vi "OPC Show.vi"(7 "queue array in":refnum<queue>[](array[refnum]), 8 "Value":variant[](array[variant]), 9 "Read":u8[](array[numeric]), 11 "Ctl In":refnum<vi>[](array[refnum])) -> ()   [LabVIEW 2012]
uses:
  <vilib>/Utility/miscctls.llb/LVRowAndColumnTypeDef.ctl
  Queue VIs/Type define/element data type.ctl
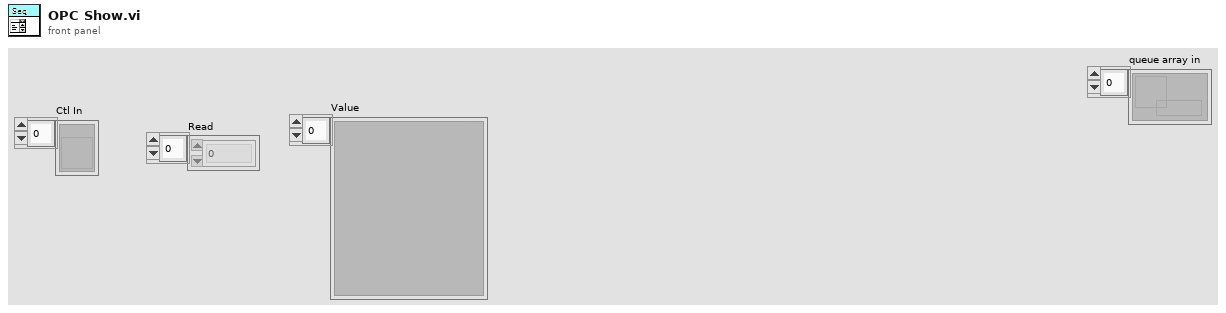
[diagram p1: front panel]
types:
  T1 = typedef "LVRowAndColumnTypeDef.ctl" = cluster{"Row":i32, "Column":i32}
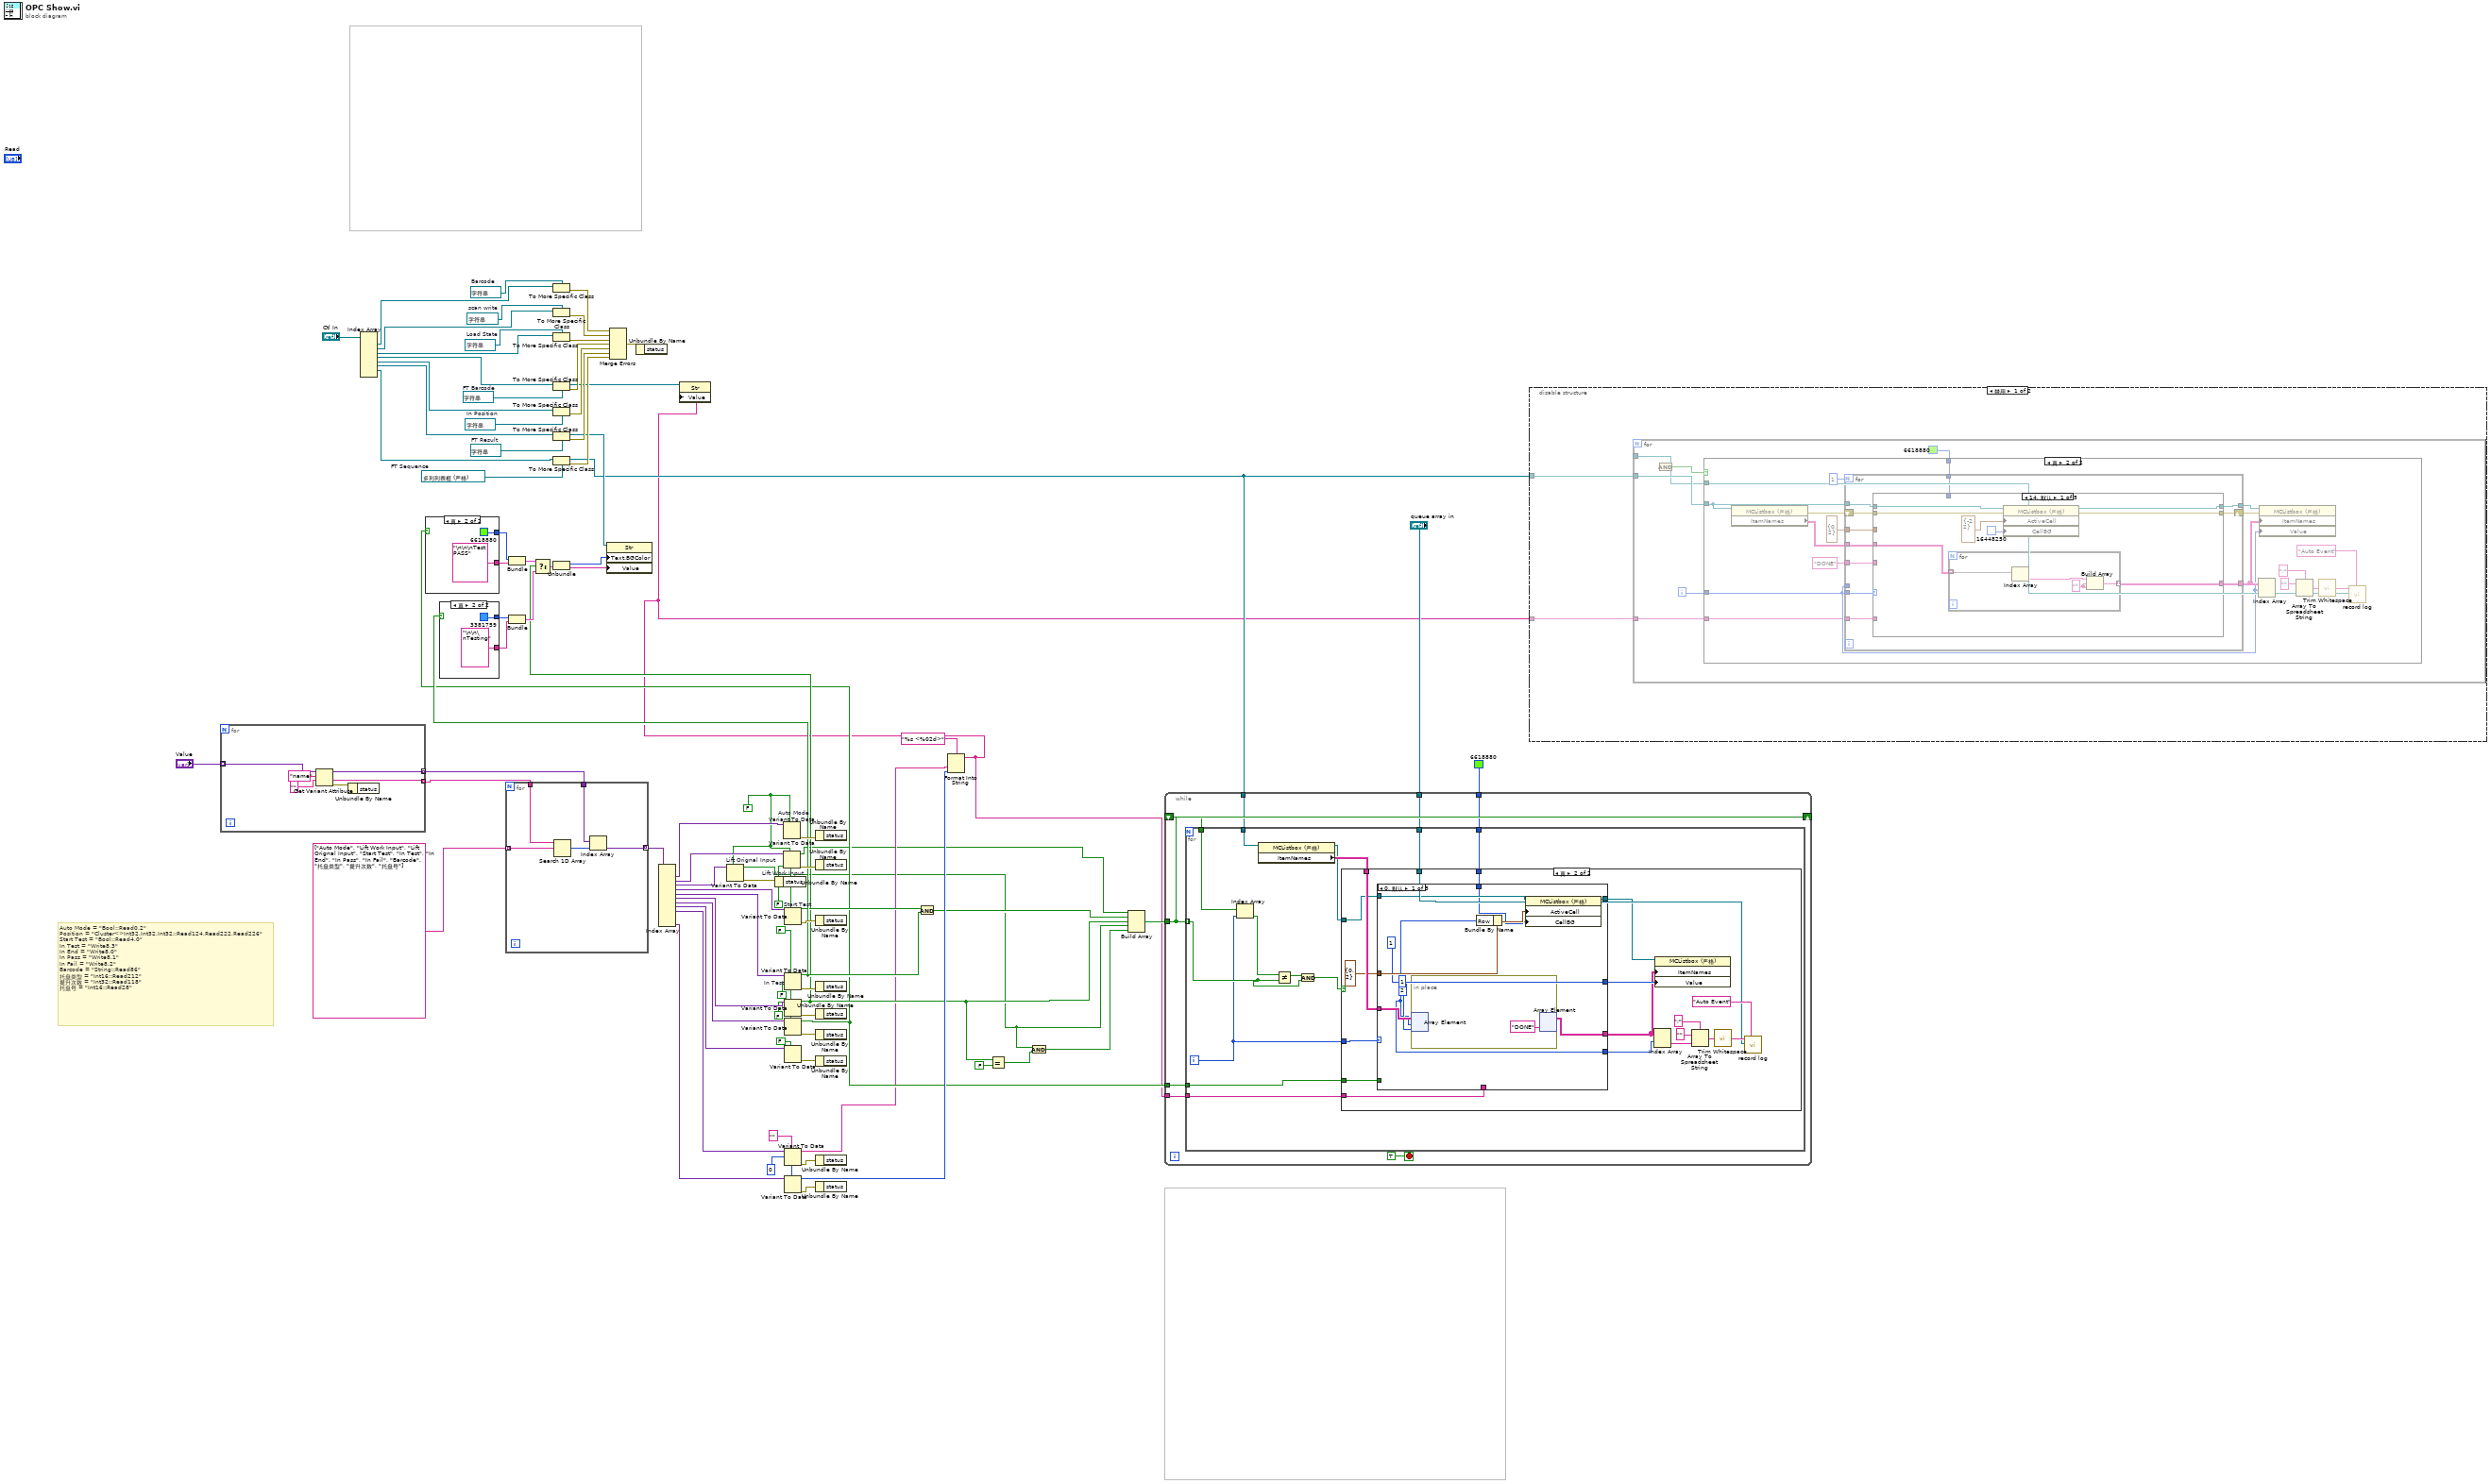
[diagram p0: block diagram]
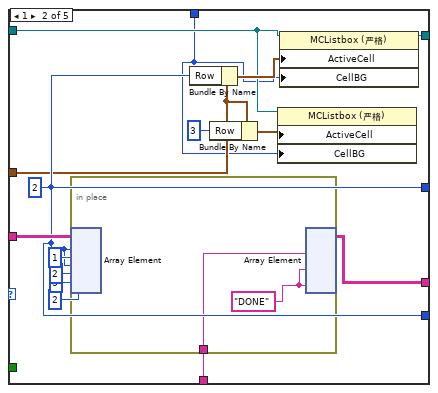
[diagram p3: hidden frame]
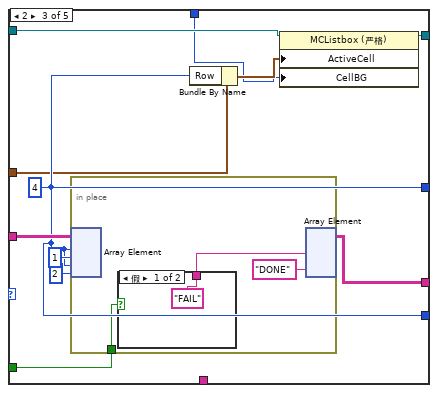
[diagram p4: hidden frame]
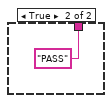
[diagram p5: hidden frame]
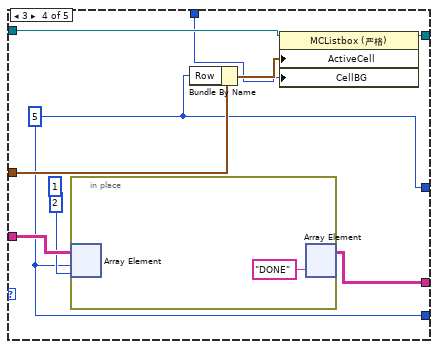
[diagram p6: hidden frame]
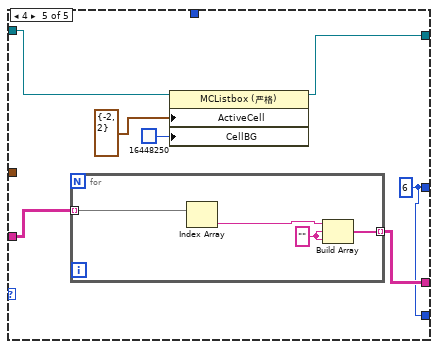
[diagram p7: hidden frame]
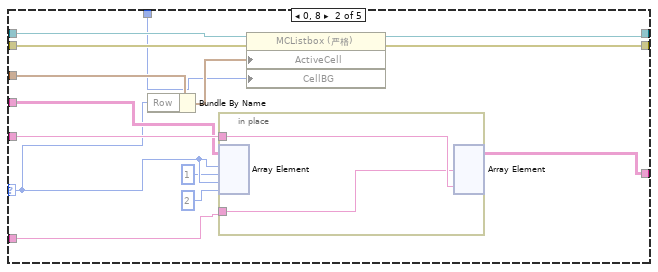
[diagram p9: hidden frame]
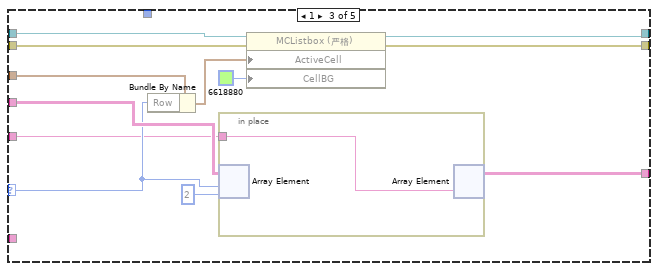
[diagram p10: hidden frame]
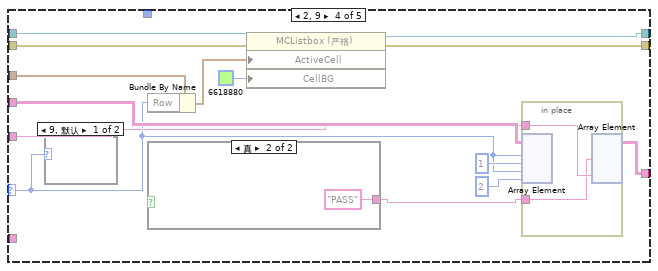
[diagram p11: hidden frame]
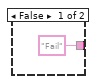
[diagram p13: hidden frame]
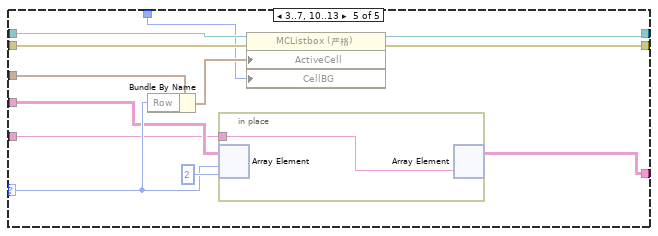
[diagram p14: hidden frame]
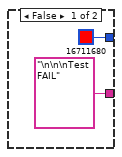
[diagram p16: hidden frame]
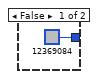
[diagram p17: hidden frame]
diagram:
  w4 = FALSE
  w77 = refnum<vi> refnum  # FT Sequence
  w78 = refnum<vi> refnum  # FT Result
  w79 = refnum<vi> refnum  # In Position
  w80 = refnum<vi> refnum  # FT Barcode
  w81 = refnum<vi> refnum  # Load State
  w82 = refnum<vi> refnum  # scan write
  w83 = refnum<vi> refnum  # Barcode
  # "Auto Mode = \"Bool::Read0.2\"\nPosition = \"Cluster<>Int32,Int32,Int32::Read124,Read222,Read226\"\nStart Test = \"Bool::Read4.0\"\nIn Test = \"Write8.3\"\nIn End = \"Write8.0\"\nIn Pass = \"Write8.1\"\nIn Fail = \"Write8.2\"\nBarcode = \"String::Read86\"\n托盘类型 = \"Int16::Read212\"\n提升次数 = \"Int32::Read118\"\n托盘号 = \"Int16::Read28\""
  n1 = for {
    tunnel: "Value" -> [w91] mode=indexing
    tunnel: [w88] -> w52 mode=indexing
    tunnel: [w86] -> w53 mode=indexing
    n2 = Get Variant Attribute(Variant=w91, name="name" ("名称"), default value (empty Variant)="" ("名称")) -> (duplicate Variant=w86:variant, value=w88:string, error out=w87:errorcluster)  [unwired: 1 in, 1 out]
    n3 = Unbundle By Name(w87) -> ()  [unwired: 1 out]
  }
  n4 = Index Array(array="Ctl In") -> (element #1=w84:refnum<vi>, element #2=w76:refnum<vi>, element #3=w75:refnum<vi>, element #4=w25:refnum<vi>, element #5=w24:refnum<vi>, element #6=w23:refnum<vi>, element #7=w22:refnum<vi>)  [unwired: 8 in, 1 out]
  n5 = for {
    tunnel: string[] ["Auto Mode", "Lift Work Input", "Lift Orignal Input", "Start Test", "In Test", "In End", "In Pass", "In Fail", "Barcode", "托盘类型", "提升次数", "托盘号"] -> [w95] mode=indexing
    tunnel: w53 -> [w94]
    tunnel: w52 -> [w96]
    tunnel: [w92] -> w51 mode=indexing
    n6 = Search 1D Array(1D array=w96, element=w95) -> (index of element=w93:i32)  [unwired: 1 in]
    n7 = Index Array(array=w94, index=w93) -> (element=w92:variant)
  }
  n8 = To More Specific Class(target class=w83, reference=w84) -> (error out=w74:errorcluster)  [unwired: 1 in, 1 out]
  n9 = To More Specific Class(target class=w82, reference=w76) -> (error out=w73:errorcluster)  [unwired: 1 in, 1 out]
  n10 = To More Specific Class(target class=w81, reference=w75) -> (error out=w72:errorcluster)  [unwired: 1 in, 1 out]
  n11 = To More Specific Class(target class=w80, reference=w25) -> (specific class reference=w67:refnum<vi>, error out=w71:errorcluster)  [unwired: 1 in]
  n12 = To More Specific Class(target class=w79, reference=w24) -> (error out=w70:errorcluster)  [unwired: 1 in, 1 out]
  n13 = To More Specific Class(target class=w78, reference=w23) -> (specific class reference=w56:refnum<vi>, error out=w69:errorcluster)  [unwired: 1 in]
  n14 = To More Specific Class(target class=w77, reference=w22) -> (specific class reference=w13:refnum<vi>, error out=w68:errorcluster)  [unwired: 1 in]
  n15 = Merge Errors(w74, w73, w72, w71, w70, w69, w68) -> (w26:errorcluster)
  n16 = Unbundle By Name(w26) -> ()  [unwired: 1 out]
  n17 = Index Array(array=w51) -> (element #1=w7:variant, element #2=w6:variant, element #3=w5:variant, element #4=w48:variant, element #5=w45:variant, element #6=w43:variant, element #7=w40:variant, element #8=w39:variant, element #9=w37:variant, element #12=w36:variant)  [unwired: 12 in, 2 out]
  n18 = Variant To Data "Lift Orignal Input"(type=w4, Variant=w5) -> (data=w1:bool, error out=w3:errorcluster)  [unwired: 1 in]
  n19 = Unbundle By Name(w3) -> ()  [unwired: 1 out]
  n20 = Variant To Data "Auto Mode"(type=w4, Variant=w7) -> (error out=w50:errorcluster)  [unwired: 1 in, 1 out]
  n21 = Variant To Data "Lift Work Input"(type=w4, Variant=w6) -> (data=w2:bool, error out=w49:errorcluster)  [unwired: 1 in]
  n22 = Variant To Data "Start Test"(type=FALSE, Variant=w48) -> (data=w20:bool, error out=w33:errorcluster)  [unwired: 1 in]
  n23 = Variant To Data "In Test"(type=FALSE, Variant=w45) -> (data=w21:bool, error out=w32:errorcluster)  [unwired: 1 in]
  n24 = case shown="真" w21 {
    tunnel: [_ "\n\n\nTesting"] -> w61
    tunnel: [u32 12369084 u32 3381759] -> w62
    frame False {
    }
    frame True {
    }
  }
  n25 = Bundle(w62, w61) -> (w63:cluster{u32, string})  [unwired: 1 in]
  n26 = Variant To Data(type=FALSE, Variant=w43) -> (data=w17:bool, error out=w31:errorcluster)  [unwired: 1 in]
  n27 = Variant To Data(type=FALSE, Variant=w40) -> (data=w10:bool, error out=w30:errorcluster)  [unwired: 1 in]
  n28 = case shown="真" w10 {
    tunnel: ["\n\n\nTest FAIL" "\n\n\nTest PASS"] -> w65
    tunnel: [u32 16711680 u32 6618880] -> w66
    frame False {
    }
    frame True {
    }
  }
  n29 = Bundle(w66, w65) -> (w64:cluster{u32, string})  [unwired: 1 in]
  n30 = Select(t=w64, s=w17, f=w63) -> (s? t:f=w60:cluster{u32, string})
  n31 = Unbundle(w60) -> (w59:u32, w58:string)
  n32 = property class="Str"(reference=w56, "Text.BGColor"=w59, "Value"=w58) -> ()  [unwired: 1 in, 2 out]
  n33 = Variant To Data(type=FALSE, Variant=w39) -> (error out=w29:errorcluster)  [unwired: 1 in, 1 out]
  n34 = Variant To Data(type="", Variant=w37) -> (data=w9:string, error out=w28:errorcluster)  [unwired: 1 in]
  n35 = Variant To Data(type=0, Variant=w36) -> (data=w34:i32, error out=w27:errorcluster)  [unwired: 1 in]
  n36 = Unbundle By Name(w50) -> ()  [unwired: 1 out]
  n37 = Unbundle By Name(w49) -> ()  [unwired: 1 out]
  n38 = Unbundle By Name(w33) -> ()  [unwired: 1 out]
  n39 = Unbundle By Name(w32) -> ()  [unwired: 1 out]
  n40 = Unbundle By Name(w31) -> ()  [unwired: 1 out]
  n41 = Unbundle By Name(w30) -> ()  [unwired: 1 out]
  n42 = Unbundle By Name(w29) -> ()  [unwired: 1 out]
  n43 = Unbundle By Name(w28) -> ()  [unwired: 1 out]
  n44 = Unbundle By Name(w27) -> ()  [unwired: 1 out]
  n45 = And(x=w20, y=w21) -> (x .and. y?=w18:bool)
  n46 = Format Into String(format string="%s <%02d>", w9, w34) -> (resulting string=w8:string)  [unwired: 2 in, 1 out]
  n47 = property class="Str"(reference=w67, "Value"=w8) -> ()  [unwired: 1 in, 2 out]
  n48 = Equal?(x=w17, y=FALSE) -> (x = y?=w16:bool)
  n49 = And(x=w1, y=w16) -> (x .and. y?=w15:bool)
  n50 = Build Array(w2, w18, w17, w1, w15) -> (w14:bool[])
  n51 = while {
    tunnel: w14 -> [w110]
    shift-right: [w110] -> _
    shift-left: _ -> [w109]
    tunnel: w13 -> [w108]
    tunnel: "queue array in" -> [w107]
    tunnel: u32 6618880 -> [w106]
    tunnel: w10 -> [w105]
    tunnel: w8 -> [w104]
    stop <- TRUE stop-if-true
    n52 = for {
      tunnel: w110 -> [w123] mode=indexing
      tunnel: w109 -> [w120]
      tunnel: w108 -> [w118]
      tunnel: w107 -> [w116]
      tunnel: w106 -> [w114]
      tunnel: w105 -> [w113]
      tunnel: w104 -> [w112]
      i -> [w121]
      n53 = Index Array(array=w120, index=w121) -> (element=w119:bool)
      n54 = property on="Property Node" class="MCListbox (严格)"(reference=w118) -> (reference out=w115:refnum<vi>, "ItemNames"=w117:string[][])  [unwired: 1 in, 1 out]
      n55 = Not Equal?(x=w119, y=w123) -> (x != y?=w124:bool)
      n56 = And(x=w124, y=w123) -> (x .and. y?=w122:bool)
      n57 = case shown="真" w122 {
        tunnel: w121 -> [_ w142]
        tunnel: w117 -> [_ w133]
        tunnel: w116 -> [_ w136]
        tunnel: w115 -> [_ w131]
        tunnel: w114 -> [_ w128]
        tunnel: w113 -> [_ w126]
        tunnel: w112 -> [_ w125]
        frame False {
        }
        frame True {
          n58 = case shown="0, 默认" w142 {
            tunnel: [w143 w161 w174 w186 w196] -> w134
            tunnel: w133 -> [w151 w167 w180 w194 w197]
            tunnel: [w150 w166 w179 w193 w198] -> w132
            tunnel: w131 -> [w148 w158 w173 w191 w200]
            tunnel: [w147 w163 w176 w190 w199] -> w130
            tunnel: T1 {"Row"=0, "Column"=2} ("Active Cell:Active Cell") -> [w146 w157 w172 w189 _]
            tunnel: w128 -> [w144 w154 w171 w187 _]
            tunnel: [w143 w161 w174 w186 w196] -> w127
            tunnel: w126 -> [_ _ w170 _ _]
            tunnel: w125 -> [_ w153 _ _ _]
            frame 0, Default {
              (unwired) 1
              w143 = 1 ("值")
              n59 = in-place {
                n60 = in-place-array #1(w151, w143, 2) -> ()  [unwired: 1 out]
                n61 = in-place-array #1("DONE" ("元素")) -> (w150:string[][])  [unwired: 2 out]
              }
              n62 = Bundle By Name(cluster=w146, "Row"=w143) -> (w145:T1)
              n63 = property on="Property Node" class="MCListbox (严格)"(reference=w148, "ActiveCell"=w145, "CellBG"=w144) -> (reference out=w147:refnum<vi>)  [unwired: 1 in, 1 out]
            }
            frame 1 {
              w161 = 2 ("值")
              n64 = in-place {
                in-place-border: w153 -> [w168]
                w169 = "DONE" ("元素")
                n65 = in-place-array #2(w167, w161, 1, w161, 2, 3, 2) -> ()  [unwired: 3 out]
                n66 = in-place-array #2(w168, w169, w169) -> (w166:string[][])  [unwired: 6 out]
              }
              n67 = Bundle By Name(cluster=w157, "Row"=w161) -> (w162:T1)
              n68 = Bundle By Name(cluster=w157, "Row"=3) -> (w156:T1)
              n69 = property on="Property Node" class="MCListbox (严格)"(reference=w158, "ActiveCell"=w156, "CellBG"=w154) -> ()  [unwired: 1 in, 2 out]
              n70 = property on="Property Node" class="MCListbox (严格)"(reference=w158, "ActiveCell"=w162, "CellBG"=w154) -> (reference out=w163:refnum<vi>)  [unwired: 1 in, 1 out]
            }
            frame 2 {
              w174 = 4 ("值")
              n71 = in-place {
                in-place-border: w170 -> [w182]
                n72 = in-place-array #3(w180, w174, 1, w174, 2) -> ()  [unwired: 2 out]
                n73 = case shown="假" w182 {
                  tunnel: ["FAIL" ("元素") "PASS" ("元素")] -> w181
                  frame False {
                  }
                  frame True {
                  }
                }
                n74 = in-place-array #3(w181, "DONE" ("元素")) -> (w179:string[][])  [unwired: 4 out]
              }
              n75 = Bundle By Name(cluster=w172, "Row"=w174) -> (w175:T1)
              n76 = property on="Property Node" class="MCListbox (严格)"(reference=w173, "ActiveCell"=w175, "CellBG"=w171) -> (reference out=w176:refnum<vi>)  [unwired: 1 in, 1 out]
            }
            frame 3 {
              (unwired) 1
              w186 = 5 ("值")
              n77 = in-place {
                n78 = in-place-array #4(w194, w186, 2) -> ()  [unwired: 1 out]
                n79 = in-place-array #4("DONE" ("元素")) -> (w193:string[][])  [unwired: 2 out]
              }
              n80 = Bundle By Name(cluster=w189, "Row"=w186) -> (w188:T1)
              n81 = property on="Property Node" class="MCListbox (严格)"(reference=w191, "ActiveCell"=w188, "CellBG"=w187) -> (reference out=w190:refnum<vi>)  [unwired: 1 in, 1 out]
            }
            frame 4 {
              w196 = 6 ("值")
              n82 = for {
                tunnel: w197 -> [w205] mode=indexing
                tunnel: [w204] -> w198 mode=indexing
                w203 = "" ("element")
                n83 = Index Array(array=w205) -> (element=w206:string)  [unwired: 1 in]
                n84 = Build Array(w206, w203, w203) -> (w204:string[])
              }
              n85 = property on="Property Node" class="MCListbox (严格)"(reference=w200, "ActiveCell"=T1 {"Row"=-2, "Column"=2} ("Active Cell:Active Cell"), "CellBG"=u32 16448250) -> (reference out=w199:refnum<vi>)  [unwired: 1 in, 1 out]
            }
          }
          n86 = Index Array(array=w132, index (row)=w127) -> (element=w135:string[])  [unwired: 1 in]
          n87 = property on="Property Node" class="MCListbox (严格)"(reference=w130, "ItemNames"=w132, "Value"=w134) -> ()  [unwired: 1 in, 2 out]
          n88 = Array To Spreadsheet String(delimiter (Tab)=";", array=w135, 3:"" ("format string")) -> (spreadsheet string=w139:string)
          n89 = call <vilib>:"Trim Whitespace.vi"("string"=w139) -> ("trimmed string"=w137:string)  [unwired: 1 in]
          n90 = call "record log.vi"("Event type"="Auto Event", "queue array in"=w136, "log"=w137) -> ()  [unwired: 8 in, 1 out]
        }
      }
    }
  }
  n91 = disable-structure shown="禁用" {
    disable-tunnel: w13 -> [w209 _]
    disable-tunnel: w8 -> [w207 _]
    frame Disabled {
      n92 = for {
        tunnel: w209 -> [w215]
        tunnel: [w212] -> w208
        tunnel: w207 -> [w210]
        i -> [w213]
        n93 = And() -> (x .and. y?=w214:bool)  [unwired: 2 in]
        n94 = case shown="真" w214 {
          tunnel: w215 -> [_ w227]
          tunnel: w213 -> [_ w224]
          tunnel: w212 -> [_ w226]
          tunnel: u32 6618880 -> [_ w217]
          tunnel: w210 -> [_ w216]
          frame False {
          }
          frame True {
            n95 = property on="Property Node" class="MCListbox (严格)"(reference=w227) -> (error out=w228:errorcluster, "ItemNames"=w234:string[][])  [unwired: 1 in, 1 out]
            n96 = for {
              N: 1 -> [_]
              tunnel: w234 -> [w245]
              tunnel: [w237] -> w225
              tunnel: "DONE" ("element") -> [w244]
              tunnel: w227 -> [w243]
              tunnel: [w242] -> w232
              tunnel: T1 {"Row"=0, "Column"=2} ("Active Cell:Active Cell") -> [w241]
              shift-right: [w240] -> w230
              shift-left: w228 -> [w239]
              tunnel: w224 -> [w238]
              tunnel: w224 -> [_]
              tunnel: w217 -> [w236]
              tunnel: w216 -> [w235]
              n97 = case shown="14, 默认" w238 {
                selector: w238 -> [_ w261 w276 w287 w308]
                tunnel: w245 -> [w253 w266 w278 w293 w307]
                tunnel: [w252 w264 w277 w292 w309] -> w237
                tunnel: w244 -> [_ w270 w274 w290 w306]
                tunnel: w243 -> [w251 w263 w282 w297 w314]
                tunnel: [w248 w268 w281 w296 w313] -> w242
                tunnel: w241 -> [_ w267 w285 w300 w316]
                tunnel: w239 -> [w247 w262 w279 w294 w311]
                tunnel: [w246 w269 w280 w295 w312] -> w240
                tunnel: w236 -> [_ w259 _ _ w305]
                tunnel: w235 -> [_ w258 _ _ _]
                frame 14, Default {
                  n98 = for {
                    tunnel: w253 -> [w256] mode=indexing
                    tunnel: [w255] -> w252 mode=indexing
                    w254 = "" ("element")
                    n99 = Index Array(array=w256) -> (element=w257:string)  [unwired: 1 in]
                    n100 = Build Array(w257, w254, w254) -> (w255:string[])
                  }
                  n101 = property on="Property Node" class="MCListbox (严格)"(reference=w251, error in=w247, "ActiveCell"=T1 {"Row"=-2, "Column"=2} ("Active Cell:Active Cell"), "CellBG"=u32 16448250) -> (reference out=w248:refnum<vi>, error out=w246:errorcluster)
                }
                frame 0, 8 {
                  n102 = Bundle By Name(cluster=w267, "Row"=w261) -> (w271:T1)
                  n103 = in-place {
                    in-place-border: w270 -> [w273]
                    in-place-border: w258 -> [w272]
                    n104 = in-place-array #5(w266, w261, 1, w261, 2) -> ()  [unwired: 2 out]
                    n105 = in-place-array #5(w272, w273) -> (w264:string[][])  [unwired: 4 out]
                  }
                  n106 = property on="Property Node" class="MCListbox (严格)"(reference=w263, error in=w262, "ActiveCell"=w271, "CellBG"=w259) -> (reference out=w268:refnum<vi>, error out=w269:errorcluster)
                }
                frame 1 {
                  n107 = Bundle By Name(cluster=w285, "Row"=w276) -> (w284:T1)
                  n108 = in-place {
                    in-place-border: w274 -> [w286]
                    n109 = in-place-array #6(w278, w276, 2) -> ()  [unwired: 1 out]
                    n110 = in-place-array #6(w286) -> (w277:string[][])  [unwired: 2 out]
                  }
                  n111 = property on="Property Node" class="MCListbox (严格)"(reference=w282, error in=w279, "ActiveCell"=w284, "CellBG"=u32 6618880) -> (reference out=w281:refnum<vi>, error out=w280:errorcluster)
                }
                frame 2, 9 {
                  n112 = case shown="9, 默认" w287 {
                    frame 9, Default {
                    }
                    frame 2 {
                    }
                  }
                  n113 = Bundle By Name(cluster=w300, "Row"=w287) -> (w299:T1)
                  n114 = case shown="真" {
                    selector: _ -> [_ _]
                    tunnel: ["Fail" ("element") "PASS" ("element")] -> w288
                    frame False {
                    }
                    frame True {
                    }
                  }
                  n115 = property on="Property Node" class="MCListbox (严格)"(reference=w297, error in=w294, "ActiveCell"=w299, "CellBG"=u32 6618880) -> (reference out=w296:refnum<vi>, error out=w295:errorcluster)
                  n116 = in-place {
                    in-place-border: w290 -> [w304]
                    in-place-border: w288 -> [w303]
                    n117 = in-place-array #7(w293, w287, 1, w287, 2) -> ()  [unwired: 2 out]
                    n118 = in-place-array #7(w303, w304) -> (w292:string[][])  [unwired: 4 out]
                  }
                }
                frame 3..7, 10..13 {
                  n119 = Bundle By Name(cluster=w316, "Row"=w308) -> (w315:T1)
                  n120 = in-place {
                    in-place-border: w306 -> [w317]
                    n121 = in-place-array #8(w307, w308, 2) -> ()  [unwired: 1 out]
                    n122 = in-place-array #8(w317) -> (w309:string[][])  [unwired: 2 out]
                  }
                  n123 = property on="Property Node" class="MCListbox (严格)"(reference=w314, error in=w311, "ActiveCell"=w315, "CellBG"=w305) -> (reference out=w313:refnum<vi>, error out=w312:errorcluster)
                }
              }
            }
            n124 = Index Array(array=w225, index (row)=w224) -> (element=w223:string[])  [unwired: 1 in]
            n125 = property on="Property Node" class="MCListbox (严格)"(reference=w232, error in=w230, "ItemNames"=w225, "Value"=w224) -> ()  [unwired: 2 out]
            n126 = Array To Spreadsheet String(delimiter (Tab)=";", array=w223, 3:"" ("format string")) -> (spreadsheet string=w220:string)
            n127 = call <vilib>:"Trim Whitespace.vi"("string"=w220) -> ("trimmed string"=w218:string)  [unwired: 1 in]
            n128 = call "record log.vi"("Event type"="Auto Event", "queue array in"=w226, "log"=w218) -> ()  [unwired: 8 in, 1 out]
          }
        }
      }
    }
    frame Enabled {
    }
  }
